vi "Project_1.vi"() -> ()   [LabVIEW 2026]
panel:
  out "client server":dbl
  in  "OK Button":bool
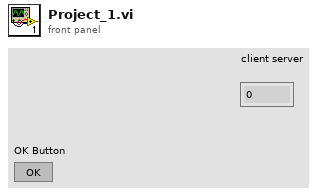
[diagram p1: front panel]
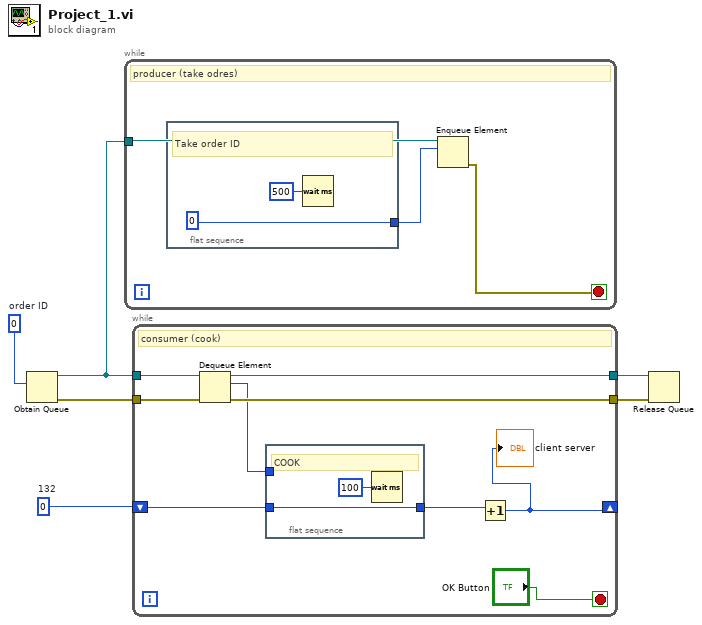
[diagram p0: block diagram]
diagram:
  w2 = 0  # 132
  w1 = 0  # order ID
  n1 = Obtain Queue(element data type=w1) -> (queue out=w6:refnum<queue>, error out=w5:errorcluster)  [unwired: 4 in, 1 out]
  n2 = while {
    tunnel: w6 -> [w8]
    stop <- w9 stop-if-true
    # "producer (take odres)"
    n3 = flat-sequence {
      tunnel: [0] -> w7
      frame #0 {
        # "Take order ID"
        n4 = Wait (ms)(milliseconds to wait=u32 500) -> ()  [unwired: 1 out]
      }
    }
    n5 = Enqueue Element(queue=w8, element=w7) -> (error out=w9:errorcluster)  [unwired: 2 in, 2 out]
  }
  n6 = while {
    tunnel: w6 -> [w19]
    tunnel: w5 -> [w20]
    tunnel: [w18] -> w4
    tunnel: [w17] -> w3
    shift-right: [w12] -> _
    shift-left: w2 -> [w16]
    stop <- "OK Button" stop-if-true
    # "consumer (cook)"
    n7 = Dequeue Element(queue=w19, error in (no error)=w20) -> (queue out=w18:refnum<queue>, element=w15:i32, error out=w17:errorcluster)  [unwired: 1 in, 1 out]
    n8 = flat-sequence {
      tunnel: w16 -> [w22]
      tunnel: [w22] -> w14
      tunnel: w15 -> [_]
      frame #0 {
        # "COOK"
        n9 = Wait (ms)(milliseconds to wait=u32 100) -> ()  [unwired: 1 out]
      }
    }
    n10 = Increment(x=w14) -> (x+1=w12:i32)
    "client server" <- w12
  }
  n11 = Release Queue(queue=w4, error in (no error)=w3) -> ()  [unwired: 1 in, 3 out]
